vi "Phase2_SCADA_Core_copy.vi"() -> ()   [LabVIEW 2026]
uses:
  SCADA_Tags.ctl
  <vilib>/sound2/lvsound2.llb/Sound Input Read (DBL).vi
  <vilib>/express/express analysis/Spectral/Block/exnSpectralBlock spectral measurements RMS poly.vi
  <vilib>/express/express analysis/Spectral/Block/exnSpectralBlock spectral measurements RMS array WFM.vi
  <vilib>/express/express analysis/Spectral/XNode/ExpressSpectralMeasurementsBlockNode.xnode
  <vilib>/Analysis/NI_AALPro.lvlib
  <vilib>/Analysis/NI_AAL_SigProc.lvlib
panel:
  in  "offkey_tol":dbl=0.3
  out "BPM":dbl(knob) scale=40.0..220.0
  in  "BPM_Max":dbl=160.0
  in  "BPM_Min":dbl=80.0
  in  "dB_Threshold":dbl=-3.0
  in  "stop 3":bool
  in  "stop 2":bool
  out "Name":string
  out "Detected Pitch(Hz)":dbl
  out "Loudness(dB)":dbl(slide) scale=-60.0..10.0
  out "Frequency Spectrum":cluster{"f0":dbl, "df":dbl, "magnitude":dbl[]}[](graph)
  out "Waveform Chart":waveform(dbl)[](graph)
  in  "stop":bool
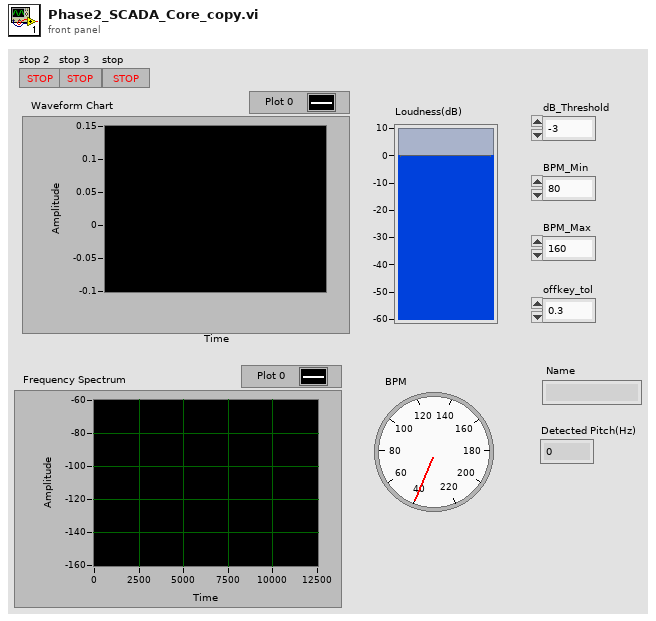
[diagram p1: front panel]
types:
  T1 = enum16{"open", "replace", "create", "open or create", "replace or create", "replace or create with confirmation"}
  T2 = typedef "SCADA_Tags.ctl" = cluster{"BPM":dbl, "dB_Level":dbl, "Pitch_Hz":dbl, "Note Name":string, "Alarm_Clipping":bool, "Alarm_Tempo":bool, "Alarm_Offkey":bool, "System_Running":bool}
  T3 = typedef "Sound Input Task ID.ctl" = u32
  T4 = cluster{"averaging mode":u16, "weighting mode":u16, "number of averages":u32}
  T5 = cluster{"dB On (F)":bool, "unwrap phase (F)":bool, "convert to degree (F)":bool}
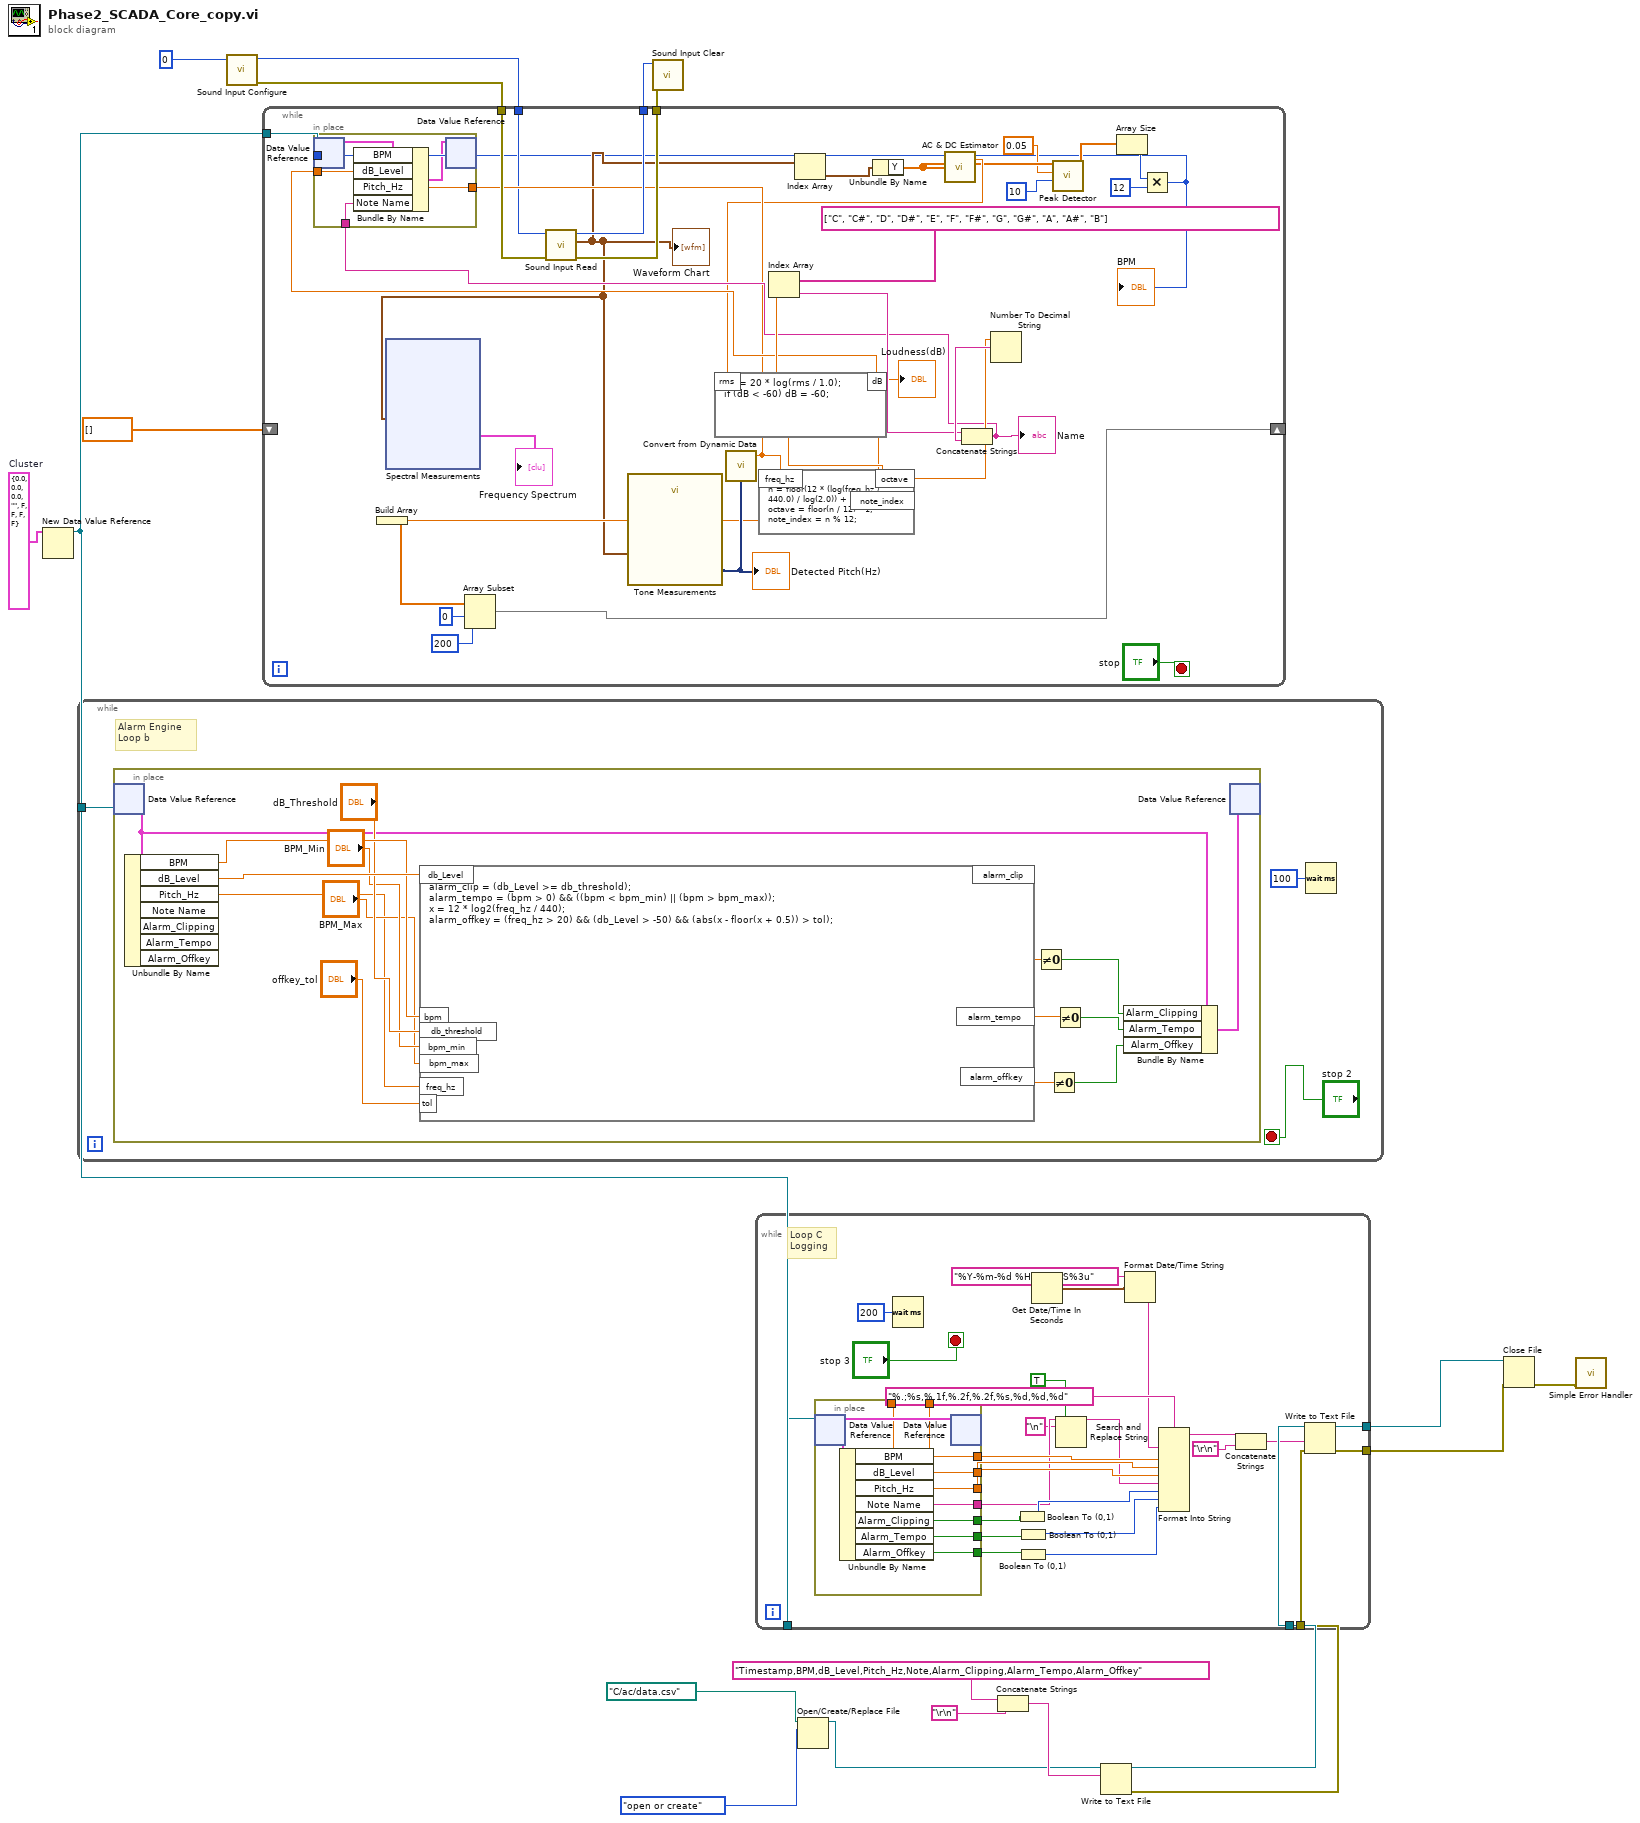
[diagram p0: block diagram]
diagram:
  w14 = T2 {"BPM"=0.0, "dB_Level"=0.0, "Pitch_Hz"=0.0, "Note Name"="", "Alarm_Clipping"=FALSE, "Alarm_Tempo"=FALSE, "Alarm_Offkey"=FALSE, "System_Running"=FALSE}  # Cluster
  n1 = New Data Value Reference(data value=w14) -> (data value reference=w13:refnum<data-value>)  [unwired: 1 in, 1 out]
  n2 = while {
    tunnel: w13 -> [w21]
    stop <- "stop 2" stop-if-true
    # "Alarm Engine \nLoop b"
    n3 = in-place {
      n4 = in-place-dvr #1(w21) -> (w27:T2)  [unwired: 1 out]
      n5 = Unbundle By Name(w27) -> ("BPM"=w36:dbl, "dB_Level"=w37:dbl, "Pitch_Hz"=w31:dbl)  [unwired: 4 out]
      n6 = formula code="float64 x;\nalarm_clip = (db_Level >= db_threshold);\nalarm_tempo = (bpm > 0) && ((bpm < bpm_min) || (bpm > bpm_max));\nx = 12 * log2(freq_hz / 440);\nalarm_offkey = (freq_hz > 20) && (db_Level > -50) && (abs(x - floor(x + 0.5)) > tol);"("db_Level"=w37, "bpm"=w36, "db_threshold"="dB_Threshold", "bpm_min"="BPM_Min", "bpm_max"="BPM_Max", "freq_hz"=w31, "tol"="offkey_tol") -> ("alarm_clip"=w30:dbl, "alarm_tempo"=w29:dbl, "alarm_offkey"=w28:dbl)
      n7 = Not Equal To 0?(x=w30) -> (x != 0?=w25:bool)
      n8 = Not Equal To 0?(x=w28) -> (x != 0?=w23:bool)
      n9 = Not Equal To 0?(x=w29) -> (x != 0?=w24:bool)
      n10 = Bundle By Name(cluster=w27, "Alarm_Clipping"=w25, "Alarm_Tempo"=w24, "Alarm_Offkey"=w23) -> (w26:T2)
      n11 = in-place-dvr #1(w26) -> ()  [unwired: 2 out]
    }
    n12 = Wait (ms)(milliseconds to wait=u32 100) -> ()  [unwired: 1 out]
  }
  n13 = call <vilib>:"Sound Input Configure.vi"("device ID"=0) -> ("error out"=w19:errorcluster, "task ID"=w18:T3)  [unwired: 9 in]
  n14 = while {
    tunnel: w19 -> [w67]
    tunnel: w18 -> [w48]
    tunnel: [w66] -> w17
    tunnel: [w65] -> w16
    shift-right: [w53] -> _
    shift-left: dbl[] [] -> [_]
    tunnel: w13 -> [w52]
    stop <- "stop" stop-if-true
    n15 = call-poly <vilib>:"Sound Input Read.vi"("error in (no error)"=w67, "task ID"=w48) -> ("error out"=w65:errorcluster, "data"=w46:waveform(dbl)[], "task ID out"=w66:T3)  [unwired: 7 in]
    "Waveform Chart" <- w46
    n16 = xnode "Spectral Measurements"("Signals"=w46) -> ("FFT - (RMS)"=→"Frequency Spectrum":cluster{"f0":dbl, "df":dbl, "magnitude":dbl[]}[])  [unwired: 1 in, 2 out]
    n17 = call "Tone Measurements"("Signals"=w46) -> ("Frequency"=w62:dynamicdata)  [unwired: 9 in, 1 out]
    "Detected Pitch(Hz)" <- w62
    n18 = call "Convert from Dynamic Data"("Dynamic Data Type"=w62) -> ("Scalar"=w49:dbl)  [unwired: 3 in]
    n19 = formula code="int n;\nn = floor(12 * (log(freq_hz / 440.0) / log(2.0)) + 0.5) + 57;\noctave = floor(n / 12) - 1;\nnote_index = n % 12;"("freq_hz"=w49) -> ("octave"=w60:dbl, "note_index"=w61:dbl)
    n20 = Index Array(array=string[] ["C", "C#", "D", "D#", "E", "F", "F#", "G", "G#", "A", "A#", "B"], index=w61) -> (element=w58:string)
    n21 = Index Array(array=w46) -> (element=w47:waveform(dbl))  [unwired: 1 in]
    n22 = Unbundle By Name(w47) -> ("Y"=w44:dbl[])
    n23 = call <vilib>:"AC & DC Estimator.vi"("Signal (V)"=w44) -> ("AC estimate (Vrms)"=w45:dbl)  [unwired: 1 out]
    n24 = formula code="dB = 20 * log(rms / 1.0);\nif (dB < -60) dB = -60;"("rms"=w45) -> ("dB"=w51:dbl)
    "Loudness(dB)" <- w51
    n25 = Build Array(w51) -> (w57:dbl[])
    n26 = Array Subset(array=w57, index=0, length=200) -> (w53:dbl[])
    n27 = Number To Decimal String(number=w60) -> (decimal integer string=w63:string)  [unwired: 1 in]
    n28 = Concatenate Strings(w58, w63) -> (w50:string)
    "Name" <- w50
    n29 = call <vilib>:"Peak Detector.vi"("width"=10, "threshold"=0.05, "X"=w44) -> ("Locations"=w41:dbl[])  [unwired: 4 in, 4 out]
    n30 = Array Size(array=w41) -> (size(s)=w40:i32)
    n31 = Multiply(x=w40, y=12) -> (x*y=w38:i32)
    "BPM" <- w38
    n32 = in-place {
      in-place-border: w38 -> [w71]
      in-place-border: w51 -> [w70]
      in-place-border: w50 -> [w69]
      in-place-border: w49 -> [w68]
      n33 = in-place-dvr #2(w52) -> (w73:T2)  [unwired: 1 out]
      n34 = Bundle By Name(cluster=w73, "BPM"=w71, "dB_Level"=w70, "Pitch_Hz"=w68, "Note Name"=w69) -> (w72:T2)
      n35 = in-place-dvr #2(w72) -> ()  [unwired: 2 out]
    }
  }
  n36 = call <vilib>:"Sound Input Clear.vi"("error in (no error)"=w16, "task ID"=w17) -> ()  [unwired: 9 in, 1 out]
  n37 = Open/Create/Replace File(file path (use dialog)=path "C:/ac/data.csv", operation (0:open)=T1."open or create") -> (refnum out=w1:refnum<file>)  [unwired: 4 in, 2 out]
  n38 = Concatenate Strings("Timestamp,BPM,dB_Level,Pitch_Hz,Note,Alarm_Clipping,Alarm_Tempo,Alarm_Offkey" ("string"), "\r\n") -> (w9:string)
  n39 = Write to Text File(file (use dialog)=w1, text=w9) -> (refnum out=w8:refnum<file>, error out=w7:errorcluster)  [unwired: 2 in, 1 out]
  n40 = while {
    tunnel: w13 -> [w106]
    tunnel: w8 -> [w92]
    tunnel: w7 -> [w91]
    tunnel: [w89] -> w6
    tunnel: [w88] -> w5
    stop <- "stop 3" stop-if-true
    # "Loop C\nLogging"
    n41 = in-place {
      in-place-border: [w113] -> _
      in-place-border: [w114] -> _
      in-place-border: [w117] -> w105
      in-place-border: [w116] -> w104
      in-place-border: [w115] -> w103
      in-place-border: [w114] -> w100
      in-place-border: [w113] -> w99
      in-place-border: [w112] -> w98
      in-place-border: [w111] -> w87
      n42 = in-place-dvr #3(w106) -> (w118:T2)  [unwired: 1 out]
      n43 = Unbundle By Name(w118) -> ("BPM"=w114:dbl, "dB_Level"=w113:dbl, "Pitch_Hz"=w112:dbl, "Note Name"=w111:string, "Alarm_Clipping"=w115:bool, "Alarm_Tempo"=w116:bool, "Alarm_Offkey"=w117:bool)
      n44 = in-place-dvr #3(w118) -> ()  [unwired: 2 out]
    }
    n45 = Wait (ms)(milliseconds to wait=u32 200) -> ()  [unwired: 1 out]
    n46 = Boolean To (0,1)(Boolean=w103) -> (0, 1=w97:i16)
    n47 = Boolean To (0,1)(Boolean=w104) -> (0, 1=w96:i16)
    n48 = Boolean To (0,1)(Boolean=w105) -> (0, 1=w95:i16)
    n49 = Get Date/Time In Seconds() -> (seconds since 1Jan1904=w108:timestamp)
    n50 = Search and Replace String(replace all?=TRUE ("replace all? (F)"), input string=w87, search string="\n") -> (result string=w84:string)  [unwired: 5 in, 3 out]
    n51 = Format Date/Time String(time format string (%c)="%Y-%m-%d %H:%M:%S%3u", seconds (now)=w108) -> (date/time string=w101:string)  [unwired: 1 in]
    n52 = Format Into String(format string="%.;%s,%.1f,%.2f,%.2f,%s,%d,%d,%d", w101, w100, w99, w98, w84, w97, w96, w95) -> (resulting string=w94:string)  [unwired: 2 in, 1 out]
    n53 = Concatenate Strings(w94, "\r\n") -> (w90:string)
    n54 = Write to Text File(file (use dialog)=w92, text=w90, error in=w91) -> (refnum out=w89:refnum<file>, error out=w88:errorcluster)  [unwired: 1 in, 1 out]
  }
  n55 = Close File(refnum=w6, error in=w5) -> (error out=w4:errorcluster)  [unwired: 1 out]
  n56 = call <vilib>:"Simple Error Handler.vi"("error in (no error)"=w4) -> ()  [unwired: 4 in, 5 out]
